vi "Bench Dirty Rects.vi"() -> ()   [LabVIEW 2020]
doc: "Benchmark for RemoteVI Dirty Rects.vi: two 1920x1080 U32 pixmaps that differ in three pixels, and the same pixmap against itself, each run Iterations times. Reports the average milliseconds per call and the rectangles found."
uses:
  source/RemoteVI.lvlib
panel:
  out "ms per call (identical)":dbl
  out "rects (identical)":cluster{"x":i32, "y":i32, "w":i32, "h":i32}[](array[cluster])
  out "ms per call (3 pixels changed)":dbl
  out "rects (3 pixels changed)":cluster{"x":i32, "y":i32, "w":i32, "h":i32}[](array[cluster])
  in  "Iterations":i32=50
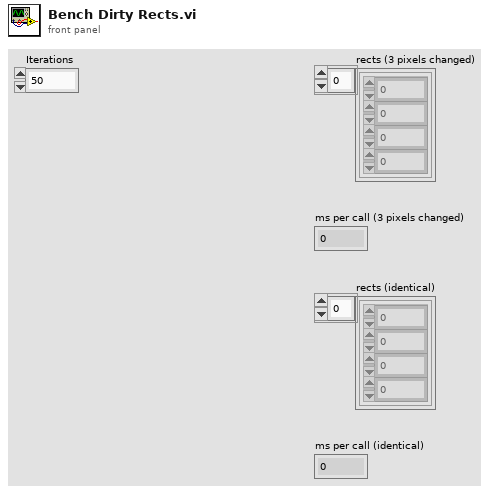
[diagram p1: front panel]
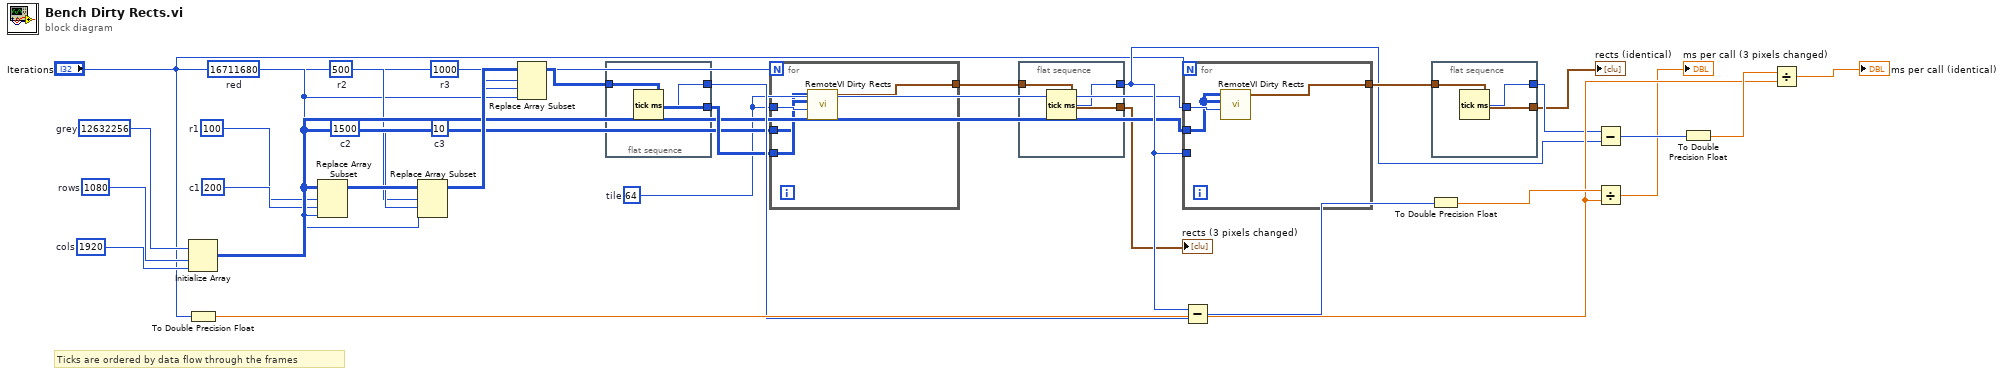
[diagram p0: block diagram]
diagram:
  w16 = 64  # tile
  w15 = 10  # c3
  w14 = 1000  # r3
  w13 = 1500  # c2
  w12 = 500  # r2
  w11 = 200  # c1
  w10 = 100  # r1
  w9 = 1920  # cols
  w8 = 1080  # rows
  w7 = u32 16711680  # red
  w6 = u32 12632256  # grey
  # "Ticks are ordered by data flow through the frames"
  n1 = Initialize Array(w6, w8, w9) -> (w17:u32[][])
  n2 = To Double Precision Float(number="Iterations") -> (double precision float=w27:dbl)
  n3 = Replace Array Subset(array=w17, new element=w7, index (row)=w10, index (col)=w11) -> (w18:u32[][])
  n4 = Replace Array Subset(array=w18, new element=w7, index (row)=w12, index (col)=w13) -> (w19:u32[][])
  n5 = Replace Array Subset(array=w19, new element=w7, index (row)=w14, index (col)=w15) -> (w20:u32[][])
  n6 = flat-sequence {
    tunnel: [w32] -> w22
    tunnel: w20 -> [w33]
    tunnel: [w33] -> w21
    frame #0 {
      n7 = Tick Count (ms)() -> (millisecond timer value=w32:u32)
    }
  }
  n8 = for {
    N: "Iterations" -> [_]
    tunnel: w16 -> [w36]
    tunnel: w17 -> [w34]
    tunnel: w21 -> [w35]
    tunnel: [w37] -> w23
    n9 = call "RemoteVI Dirty Rects.vi"("tile size"=w36, "current"=w35, "previous"=w34) -> ("rects"=w37:cluster{"x":i32, "y":i32, "w":i32, "h":i32}[])  [unwired: 8 in]
  }
  n10 = flat-sequence {
    tunnel: [w38] -> w24
    tunnel: w23 -> [w39]
    tunnel: [w39] -> w2
    frame #0 {
      n11 = Tick Count (ms)() -> (millisecond timer value=w38:u32)
    }
  }
  n12 = for {
    N: "Iterations" -> [_]
    tunnel: w16 -> [w41]
    tunnel: w17 -> [w40]
    tunnel: w24 -> [_]
    tunnel: [w42] -> w25
    n13 = call "RemoteVI Dirty Rects.vi"("tile size"=w41, "current"=w40, "previous"=w40) -> ("rects"=w42:cluster{"x":i32, "y":i32, "w":i32, "h":i32}[])  [unwired: 8 in]
  }
  n14 = Subtract(x=w24, y=w22) -> (x-y=w28:u32)
  n15 = flat-sequence {
    tunnel: [w43] -> w26
    tunnel: w25 -> [w44]
    tunnel: [w44] -> w4
    frame #0 {
      n16 = Tick Count (ms)() -> (millisecond timer value=w43:u32)
    }
  }
  n17 = To Double Precision Float(number=w28) -> (double precision float=w29:dbl)
  n18 = Subtract(x=w26, y=w24) -> (x-y=w30:u32)
  n19 = Divide(x=w29, y=w27) -> (x/y=→"ms per call (3 pixels changed)":dbl)
  n20 = To Double Precision Float(number=w30) -> (double precision float=w31:dbl)
  n21 = Divide(x=w31, y=w27) -> (x/y=→"ms per call (identical)":dbl)
  "rects (3 pixels changed)" <- w2
  "rects (identical)" <- w4
